vi "VIH UI - Undo Focused Control - Core.vi"(6 "cmd (save)":enum16{"Init", "status", "save", "undo", "redo"}(ring)=enum."save", 8 "error in":errorcluster, 10 "Need Selection (F)":bool, 11 "Ctl Refnum":refnum<vi>) -> (0 "no error out":errorcluster, 2 "Status":T1, 3 "dup Ctl Refnum":refnum<vi>)   [LabVIEW 2014]
doc: "::: VI Helpeks :::\nCopyright (c) 2000-2026 Konstantin Shifershteyn. All rights reserved."
uses:
  <vilib>/Utility/miscctls.llb/LVSelectionTypeDef.ctl
panel:
  # "VI Helpeks\nCopyright (c) 2012-2026 Konstantin Shifershteyn"
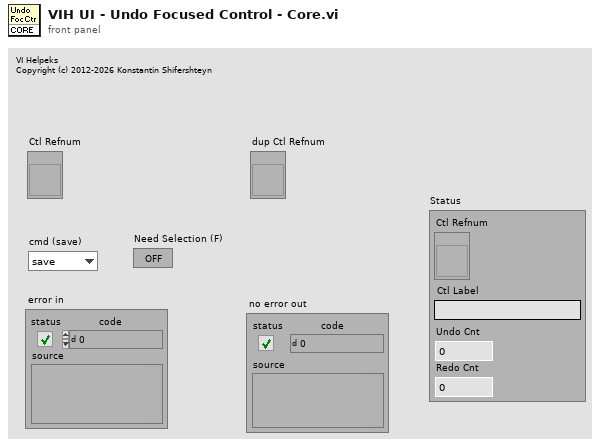
[diagram p1: front panel]
types:
  T1 = cluster{"Ctl Refnum":refnum<vi>, "Ctl Label":string, "Undo Cnt":dbl, "Redo Cnt":dbl}
  T2 = typedef "LVSelectionTypeDef.ctl" = cluster{"Selection Start":u32, "Selection End":u32}
  T3 = cluster{"Ctl Refnum":refnum<vi>, "Ctl Label":string, "Undo Buf":cluster{"Text.Text":string, "Text.Selection":T2}[], "Redo Buf":cluster{"Text.Text":string, "Text.Selection":T2}[]}
  T4 = cluster{"Text.Text":string, "Text.Selection":T2}[]
  T5 = cluster{"Ctl Refnum":refnum<vi>, "Ctl Label":string, i32, i32}
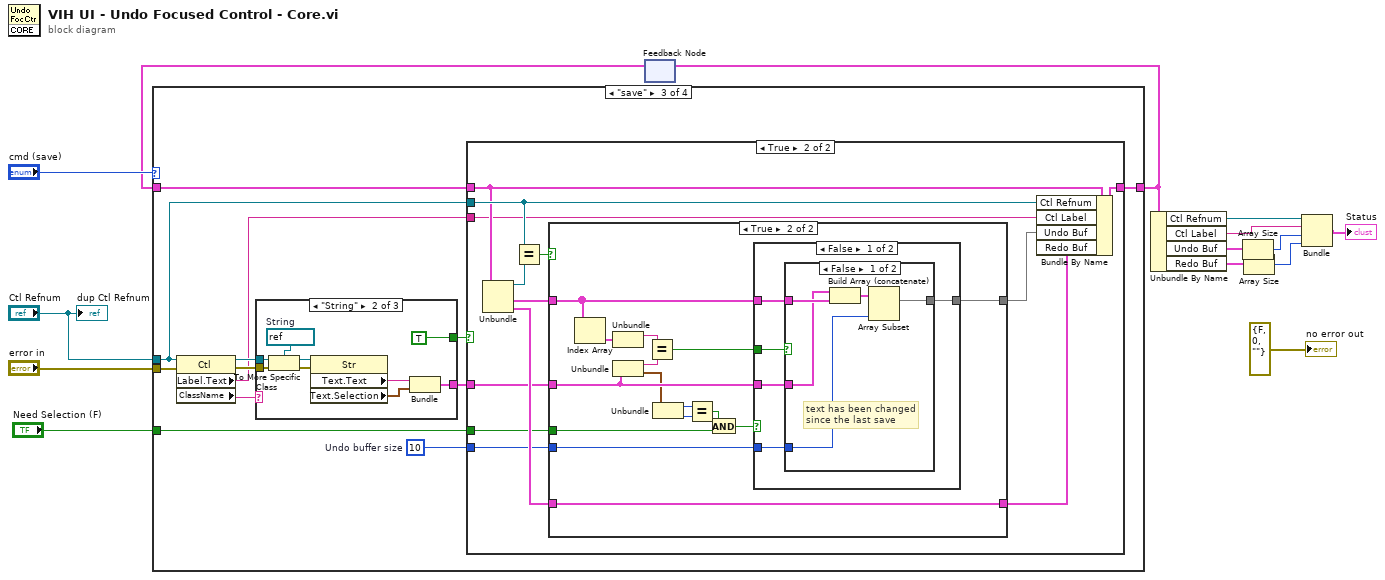
[diagram p0: block diagram]
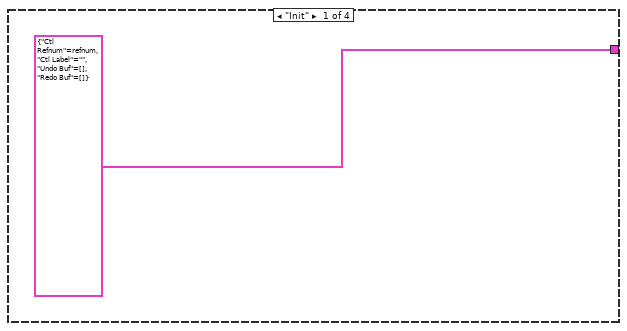
[diagram p2: hidden frame]
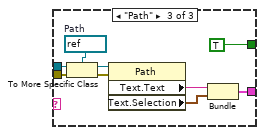
[diagram p5: hidden frame]
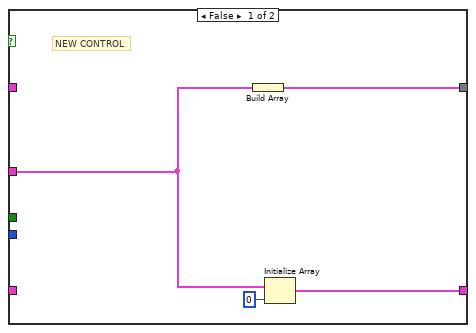
[diagram p7: hidden frame]
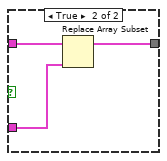
[diagram p8: hidden frame]
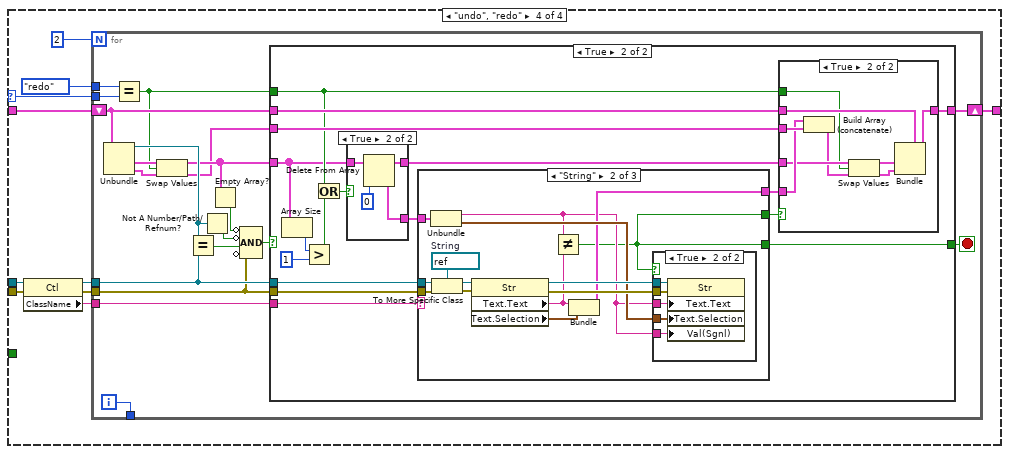
[diagram p10: hidden frame]
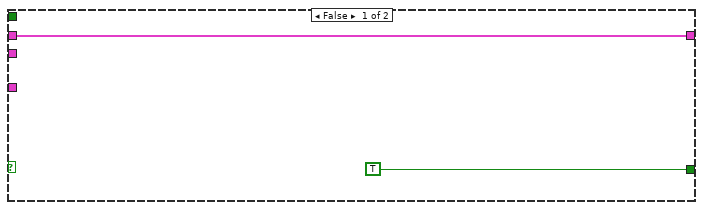
[diagram p11: hidden frame]
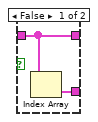
[diagram p12: hidden frame]
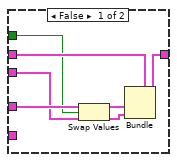
[diagram p13: hidden frame]
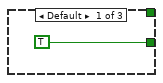
[diagram p14: hidden frame]
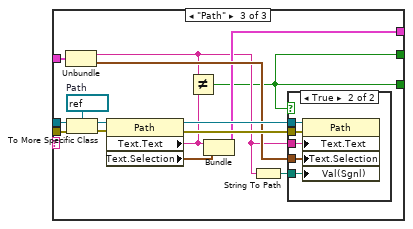
[diagram p16: hidden frame]
diagram:
  n1 = feedback #1() -> (w13:T3)  [unwired: 1 in]
  n2 = case shown="\"save\"" "cmd (save)" {
    selector: "cmd (save)" -> [_ _ _ w100]
    tunnel: "Ctl Refnum" -> [_ _ w26 w99]
    tunnel: [T3 {"Ctl Refnum"=refnum, "Ctl Label"="", "Undo Buf"=[], "Redo Buf"=[]} w16 w19 w102] -> w5
    tunnel: w13 -> [_ w16 w27 w103]
    tunnel: "error in" -> [_ _ w28 w98]
    tunnel: "Need Selection (F)" -> [_ _ w17 _]
    frame "Init" {
    }
    frame "status" {
    }
    frame "save" {
      w18 = 10  # Undo buffer size
      n3 = property class="Ctl"(reference=w26, error in=w28) -> (reference out=w25:refnum<vi>, error out=w23:errorcluster, "Label.Text"=w20:string, "ClassName"=w24:string)
      n4 = case shown="\"String\"" w24 {
        tunnel: w25 -> [_ w32 w41]
        tunnel: w23 -> [_ w31 w40]
        tunnel: [_ w30 w39] -> w22
        tunnel: [_ TRUE TRUE] -> w21
        frame Default {
        }
        frame "String" {
          w34 = refnum<vi> refnum  # String
          n5 = To More Specific Class(target class=w34, reference=w32, error in=w31) -> (specific class reference=w33:refnum<vi>, error out=w37:errorcluster)
          n6 = property class="Str"(reference=w33, error in=w37) -> ("Text.Text"=w35:string, "Text.Selection"=w36:T2)  [unwired: 2 out]
          n7 = Bundle("Text.Text"=w35, "Text.Selection"=w36) -> (w30:cluster{"Text.Text":string, "Text.Selection":T2})  [unwired: 1 in]
        }
        frame "Path" {
          w43 = refnum<vi> refnum  # Path
          n8 = To More Specific Class(target class=w43, reference=w41, error in=w40) -> (specific class reference=w42:refnum<vi>, error out=w46:errorcluster)
          n9 = property class="Path"(reference=w42, error in=w46) -> ("Text.Text"=w44:string, "Text.Selection"=w45:T2)  [unwired: 2 out]
          n10 = Bundle("Text.Text"=w44, "Text.Selection"=w45) -> (w39:cluster{"Text.Text":string, "Text.Selection":T2})  [unwired: 1 in]
        }
      }
      n11 = case shown="True" w21 {
        tunnel: [w47 w60] -> w19
        tunnel: w27 -> [w47 w51]
        tunnel: w26 -> [_ w57]
        tunnel: w22 -> [_ w52]
        tunnel: w20 -> [_ w50]
        tunnel: w18 -> [_ w49]
        tunnel: w17 -> [_ w48]
        frame False {
        }
        frame True {
          n12 = Unbundle(w51) -> ("Ctl Refnum"=w58:refnum<vi>, "Undo Buf"=w59:T4, "Redo Buf"=w53:T4)  [unwired: 1 out]
          n13 = Equal?(x=w57, y=w58) -> (x = y?=w56:bool)
          n14 = case shown="True" w56 {
            tunnel: w52 -> [w62 w78]
            tunnel: [w64 w79] -> w55
            tunnel: w59 -> [_ w77]
            tunnel: [w61 w65] -> w54
            tunnel: w53 -> [_ w65]
            tunnel: w49 -> [_ w76]
            tunnel: w48 -> [_ w66]
            frame False {
              # "NEW CONTROL"
              n15 = Build Array(w62) -> (w64:T4)
              n16 = Initialize Array(w62, 0 ("dimension size")) -> (w61:T4)
            }
            frame True {
              n17 = Index Array(array=w77) -> (element=w75:cluster{"Text.Text":string, "Text.Selection":T2})  [unwired: 1 in]
              n18 = Unbundle(w75) -> ("Text.Text"=w74:string)  [unwired: 1 out]
              n19 = Unbundle(w78) -> ("Text.Text"=w73:string, "Text.Selection"=w71:T2)
              n20 = Equal?(x=w74, y=w73) -> (x = y?=w72:bool)
              n21 = Unbundle(w71) -> ("Selection Start"=w70:u32, "Selection End"=w69:u32)
              n22 = Equal?(x=w70, y=w69) -> (x = y?=w68:bool)
              n23 = And(x=w68, y=w66) -> (x .and. y?=w67:bool)
              n24 = case shown="False" w67 {
                tunnel: [w84 w93] -> w79
                tunnel: w78 -> [w83 _]
                tunnel: w77 -> [w82 w93]
                tunnel: w76 -> [w81 _]
                tunnel: w72 -> [w80 _]
                frame False {
                  n25 = case shown="False" w80 {
                    tunnel: w82 -> [w89 w92]
                    tunnel: w83 -> [w86 w90]
                    tunnel: [w87 w91] -> w84
                    tunnel: w81 -> [w85 _]
                    frame False {
                      # "text has been changed\nsince the last save"
                      n26 = Build Array (concatenate)(w86, w89) -> (w88:T4)
                      n27 = Array Subset(array=w88, length=w85) -> (w87:T4)  [unwired: 1 in]
                    }
                    frame True {
                      n28 = Replace Array Subset "Replace Array Subset"(array=w92, new element=w90) -> (w91:T4)  [unwired: 1 in]
                    }
                  }
                }
                frame True {
                  # "do nothing if no selected\ntext but it's expected"
                }
              }
            }
          }
          n29 = Bundle By Name(cluster=w51, "Ctl Refnum"=w57, "Ctl Label"=w50, "Undo Buf"=w55, "Redo Buf"=w54) -> (w60:T3)
        }
      }
    }
    frame "undo", "redo" {
      n30 = property class="Ctl"(reference=w99, error in=w98) -> (reference out=w97:refnum<vi>, error out=w96:errorcluster, "ClassName"=w95:string)
      n31 = for {
        N: 2 -> [_]
        shift-right: [w117] -> w102
        shift-left: w103 -> [w118]
        tunnel: w100 -> [w110]
        tunnel: w97 -> [w108]
        tunnel: w96 -> [w107]
        tunnel: w95 -> [w106]
        tunnel: enum16{"Init", "status", "save", "undo", "redo"}."redo" ("x") -> [w105]
        tunnel: [w104] -> _
        i -> [w104]
        stop <- w115 stop-if-true
        n32 = Unbundle(w118) -> ("Ctl Refnum"=w122:refnum<vi>, "Undo Buf"=w114:T4, "Redo Buf"=w113:T4)  [unwired: 1 out]
        n33 = Equal?(x=w105, y=w110) -> (x = y?=w109:bool)
        n34 = Swap Values(12:w114, 13:w109, 14:w113) -> (1:w112:T4, 3:w111:T4)
        n35 = Equal?(x=w122, y=w108) -> (x = y?=w120:bool)
        n36 = Not A Number/Path/Refnum?(number/path/refnum=w122) -> (NaN/Path/Refnum?=w121:bool)
        n37 = Empty Array?(array=w112) -> (empty?=w116:bool)
        n38 = Compound Arithmetic op=AND(invert w116, invert w121, w120, invert w107) -> (w119:bool)
        n39 = case shown="True" w119 {
          tunnel: w107 -> [_ w132]
          tunnel: w108 -> [_ w133]
          tunnel: w118 -> [w124 w141]
          tunnel: w112 -> [_ w128]
          tunnel: [w124 w139] -> w117
          tunnel: w111 -> [_ w138]
          tunnel: [TRUE w134] -> w115
          tunnel: w109 -> [_ w130]
          tunnel: w106 -> [_ w131]
          frame False {
          }
          frame True {
            n40 = Array Size(array=w128) -> (size(s)=w127:i32)
            n41 = Greater?(x=w127, y=1) -> (0:w125:bool)
            n42 = Or(x=w130, y=w125) -> (x .or. y?=w129:bool)
            n43 = case shown="True" w129 {
              tunnel: w128 -> [w143 w147]
              tunnel: [w143 w145] -> w140
              tunnel: [w142 w144] -> w137
              frame False {
                n44 = Index Array(array=w143) -> (element=w142:cluster{"Text.Text":string, "Text.Selection":T2})  [unwired: 1 in]
              }
              frame True {
                n45 = Delete From Array(array=w147, index=0) -> (deleted portion=w144:cluster{"Text.Text":string, "Text.Selection":T2}, array with subset deleted=w145:T4)  [unwired: 1 in]
              }
            }
            n46 = case shown="\"String\"" w131 {
              tunnel: w133 -> [_ w178 w198]
              tunnel: w132 -> [_ w176 w196]
              tunnel: w137 -> [_ w171 w191]
              tunnel: [_ w168 w188] -> w136
              tunnel: [_ w165 w184] -> w135
              tunnel: [TRUE w165 w184] -> w134
              frame Default {
              }
              frame "String" {
                w177 = refnum<vi> refnum  # String
                n47 = Unbundle(w171) -> ("Text.Text"=w166:string, "Text.Selection"=w170:T2)
                n48 = To More Specific Class(target class=w177, reference=w178, error in=w176) -> (specific class reference=w175:refnum<vi>, error out=w174:errorcluster)
                n49 = property class="Str"(reference=w175, error in=w174) -> (reference out=w173:refnum<vi>, error out=w172:errorcluster, "Text.Text"=w167:string, "Text.Selection"=w169:T2)
                n50 = Not Equal?(x=w166, y=w167) -> (x != y?=w165:bool)
                n51 = Bundle("Text.Text"=w167, "Text.Selection"=w169) -> (w168:cluster{"Text.Text":string, "Text.Selection":T2})  [unwired: 1 in]
                n52 = case shown="True" w165 {
                  tunnel: w173 -> [_ w183]
                  tunnel: w172 -> [_ w182]
                  tunnel: w170 -> [_ w181]
                  tunnel: w166 -> [_ w180]
                  tunnel: w166 -> [_ w179]
                  frame False {
                  }
                  frame True {
                    n53 = property class="Str"(reference=w183, error in=w182, "Text.Text"=w180, "Text.Selection"=w181, "Val(Sgnl)"=w179) -> ()  [unwired: 2 out]
                  }
                }
              }
              frame "Path" {
                w197 = refnum<vi> refnum  # Path
                n54 = Unbundle(w191) -> ("Text.Text"=w186:string, "Text.Selection"=w190:T2)
                n55 = To More Specific Class(target class=w197, reference=w198, error in=w196) -> (specific class reference=w195:refnum<vi>, error out=w194:errorcluster)
                n56 = property class="Path"(reference=w195, error in=w194) -> (reference out=w193:refnum<vi>, error out=w192:errorcluster, "Text.Text"=w187:string, "Text.Selection"=w189:T2)
                n57 = Not Equal?(x=w186, y=w187) -> (x != y?=w184:bool)
                n58 = Bundle("Text.Text"=w187, "Text.Selection"=w189) -> (w188:cluster{"Text.Text":string, "Text.Selection":T2})  [unwired: 1 in]
                n59 = String To Path(string=w186) -> (path=w185:path)
                n60 = case shown="True" w184 {
                  tunnel: w193 -> [_ w203]
                  tunnel: w192 -> [_ w202]
                  tunnel: w190 -> [_ w201]
                  tunnel: w186 -> [_ w200]
                  tunnel: w185 -> [_ w199]
                  frame False {
                  }
                  frame True {
                    n61 = property class="Path"(reference=w203, error in=w202, "Text.Text"=w200, "Text.Selection"=w201, "Val(Sgnl)"=w199) -> ()  [unwired: 2 out]
                  }
                }
              }
            }
            n62 = case shown="True" w135 {
              tunnel: w141 -> [w152 w163]
              tunnel: w140 -> [w150 w159]
              tunnel: [w151 w162] -> w139
              tunnel: w138 -> [w149 w161]
              tunnel: w136 -> [_ w160]
              tunnel: w130 -> [w148 w155]
              frame False {
                n63 = Swap Values(12:w150, 13:w148, 14:w149) -> (1:w154:T4, 3:w153:T4)
                n64 = Bundle(cluster=w152, "Undo Buf"=w154, "Redo Buf"=w153) -> (w151:T3)  [unwired: 2 in]
              }
              frame True {
                n65 = Build Array (concatenate)(w160, w161) -> (w157:T4)
                n66 = Swap Values(12:w159, 13:w155, 14:w157) -> (1:w158:T4, 3:w156:T4)
                n67 = Bundle(cluster=w163, "Undo Buf"=w158, "Redo Buf"=w156) -> (w162:T3)  [unwired: 2 in]
              }
            }
          }
        }
      }
    }
  }
  n68 = feedback-in #1(w5) -> ()
  n69 = Unbundle By Name(w5) -> ("Ctl Refnum"=w3:refnum<vi>, "Ctl Label"=w6:string, "Undo Buf"=w7:T4, "Redo Buf"=w8:T4)
  n70 = Array Size(array=w7) -> (size(s)=w9:i32)
  n71 = Array Size(array=w8) -> (size(s)=w10:i32)
  n72 = Bundle("Ctl Refnum"=w3, "Ctl Label"=w6, w9, w10) -> (→"Status":T5)  [unwired: 1 in]
  "no error out" <- errorcluster {"status"=FALSE, "code"=0, "source"=""} ("no error out")
  "dup Ctl Refnum" <- "Ctl Refnum"
